vi "D_Check_IO.vi"(8 "error in (no error)":errorcluster, 11 "bID":u8) -> (0 "error out":errorcluster, 1 "IO_Status_bool":bool[](array[boolean]), 2 "IO_Status":u32, 3 "bID":u8, 4 "TorF":i32)   [LabVIEW 2013]
uses:
  LabVIEW2018/hpkSLMdaLV.dll
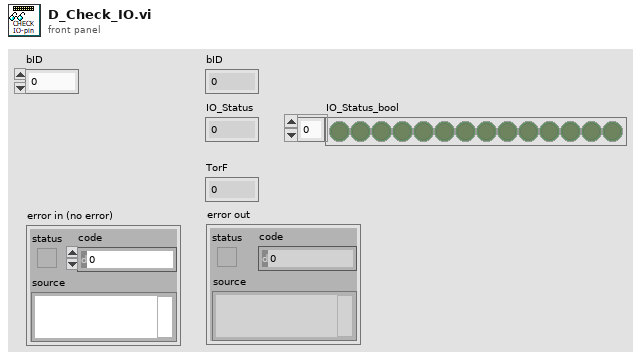
[diagram p1: front panel]
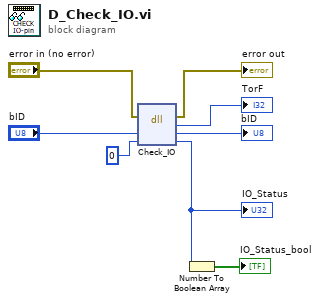
[diagram p0: block diagram]
diagram:
  n1 = dll-call lib="C:/Users/hs5921/Desktop/LabVIEW2018/hpkSLMdaLV.dll" fn="Check_IO"(error in="error in (no error)", "bID"="bID", "IO_Status"=u32 0 ("mode")) -> (error out=→"error out":errorcluster, "返り値タイプ"=→"TorF":i32, "bID"=→"bID":u8, "IO_Status"=w2:u32)  [unwired: 2 in, 1 out]
  "IO_Status" <- w2
  n2 = Number To Boolean Array(number=w2) -> (Boolean array=→"IO_Status_bool":bool[])
